vi "test tools list cache.vi"(8 "error in (no error)":errorcluster, 11 "server id":i32) -> (0 "error out":errorcluster, 3 "body":string)   [LabVIEW 2020, in "MCP Server tests.lvlib"]
doc: "Test 75: tools/list is answered from the cache and follows Add Tool.\n\nThe server builds the list of tools once and answers the following tools/list requests from Tool List Cache.vi (Cached Tool List.vi) until the tools of the server change.\n\n1. Two consecutive tools/list requests with the same id get exactly the same answer, with result.tools and without fake_tool_added_later.\n2. The second of the two, which is answered from the cache, takes less than 500 ms. The label of the assertion carries the measured time. Measured on LabVIEW 2026 with the 20 tools of this suite: 112 to 154 ms, most of it the HTTP round trip of two requests in a row.\n3. Add Tool.vi adds fake tool added later.vi to the running server; the next tools/list contains fake_tool_added_later, so the cache follows the tools.\n4. The tools/list after that gets the same answer again.\n\nThe added tool stays on the server of this test run; run this test after the tests that expect a fixed list of tools."
uses:
  MCP Server tests.lvlib
  de18a1eb-e5a6-43c2-9401-4d16a1e6fda1.vi
  a5e1876d-9ffb-455d-837e-6668acf3c3fd.vi
  <vilib>/JDP Science/JSONtext/Next JSON Value.vi
  <vilib>/JDP Science/JSONtext/String Subset.vi
  <vilib>/JDP Science/JSONtext/Parsing/Advance past next JSON Value (inlined COPY).vi
  <vilib>/JDP Science/JSONtext/Parsing/Advance past whitespace.vi
  <vilib>/JDP Science/JSONtext/Parsing/Advance past String.vi
  <vilib>/JDP Science/JSONtext/Parsing/Advance past Number.vi
  <vilib>/JDP Science/JSONtext/Parsing/Advance past Line Ending.vi
  <vilib>/JDP Science/JSONtext/Parsing/Parse Full Path or Item Name.vi
  <vilib>/JDP Science/JSONtext/Parsing/Advance past Array.vi
  <vilib>/JDP Science/JSONtext/Parsing/Advance past Object.vi
  <vilib>/JDP Science/JSONtext/support/Error Cluster From Code.vi
  <vilib>/JDP Science/JSONtext/Offset/Find Item Locations by Path.vi
  <vilib>/addons/_JKI Toolkits/Caraya/classes/Test/Test.lvclass
  <vilib>/JDP Science/JSONtext/JSONtext.lvlib
  <vilib>/addons/_JKI Toolkits/Caraya/classes/Assert/Assert.lvclass
  src/MCP Server/MCP Server.lvlib
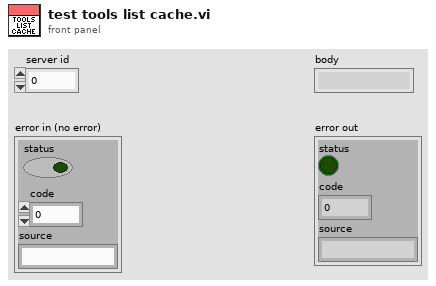
[diagram p1: front panel]
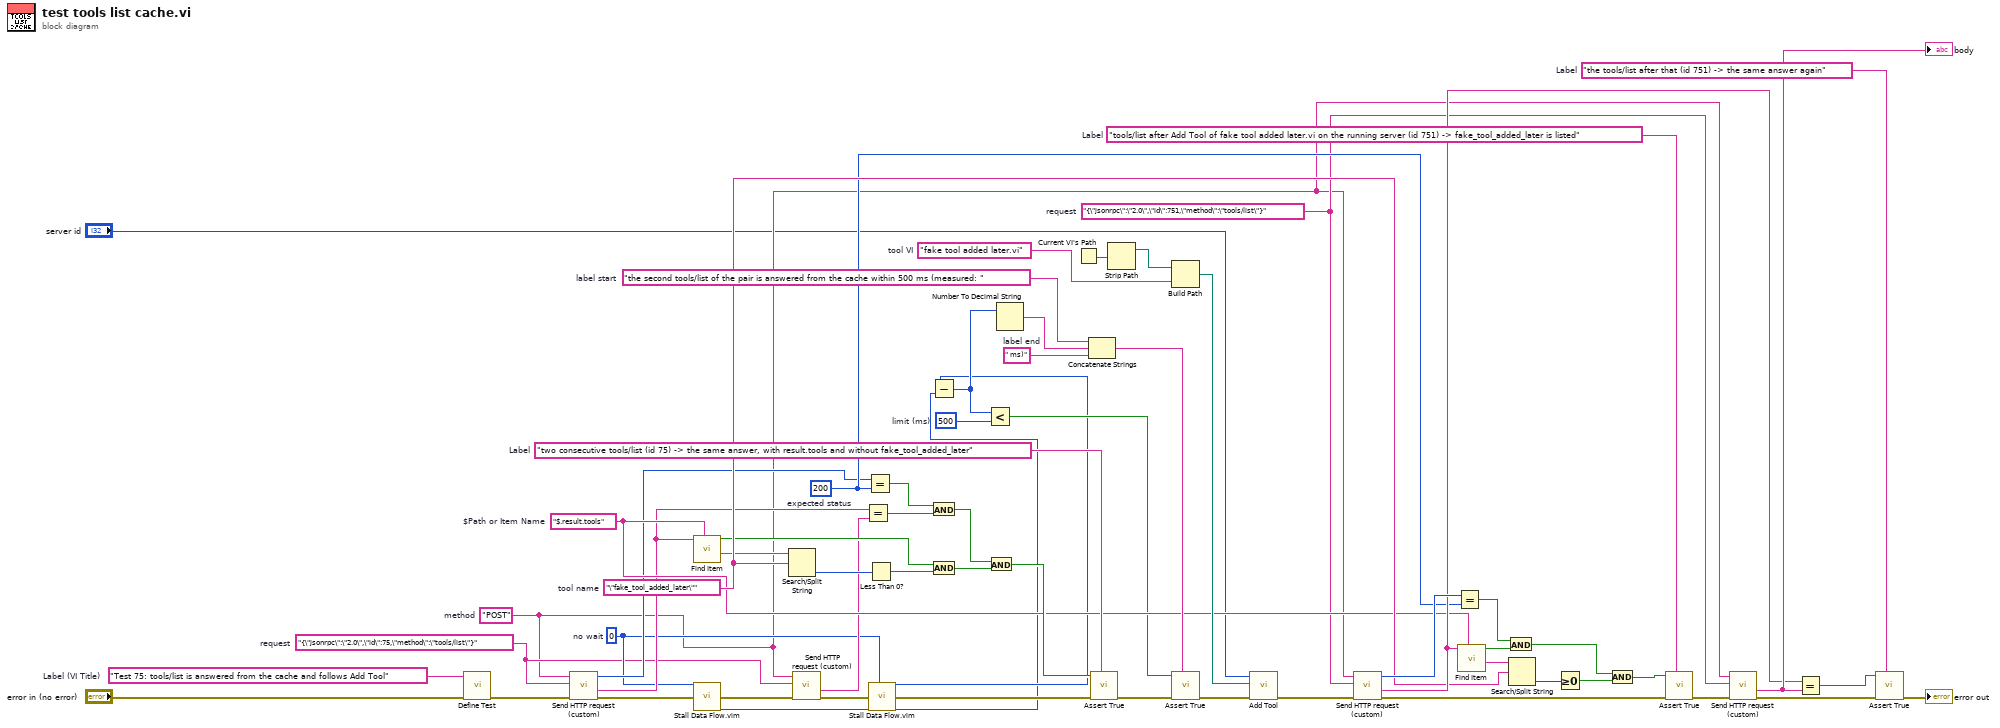
[diagram p0: block diagram]
diagram:
  w60 = "the tools/list after that (id 751) -> the same answer again"  # Label
  w55 = "tools/list after Add Tool of fake tool added later.vi on the running server (id 751) -> fake_tool_added_later is listed"  # Label
  w40 = "fake tool added later.vi"  # tool VI
  w37 = " ms)"  # label end
  w36 = "the second tools/list of the pair is answered from the cache within 500 ms (measured: "  # label start
  w33 = "two consecutive tools/list (id 75) -> the same answer, with result.tools and without fake_tool_added_later"  # Label
  w27 = "\"fake_tool_added_later\""  # tool name
  w24 = "$.result.tools"  # $Path or Item Name
  w21 = 200  # expected status
  w19 = u32 500  # limit (ms)
  w8 = 0  # no wait
  w7 = "{\"jsonrpc\":\"2.0\",\"id\":751,\"method\":\"tools/list\"}"  # request
  w6 = "{\"jsonrpc\":\"2.0\",\"id\":75,\"method\":\"tools/list\"}"  # request
  w5 = "POST"  # method
  w3 = "Test 75: tools/list is answered from the cache and follows Add Tool"  # Label (VI Title)
  n1 = call <vilib>:"Define Test.vi"("error in (no error)"="error in (no error)", "Label (VI Title)"=w3) -> ("error out"=w4:errorcluster)  [unwired: 8 in, 1 out]
  n2 = call "Send HTTP request (custom).vi"("error in (no error)"=w4, "request"=w6, "method"=w5) -> ("error out"=w9:errorcluster, "response"=w10:string, "status code"=w11:i32)  [unwired: 5 in, 1 out]
  n3 = call <vilib>:"Find Item.vi"("$Path or Item Name"=w24, "JSON"=w10) -> ("<JSON>"=w25:string, "Found"=w26:bool)  [unwired: 6 in, 2 out]
  n4 = call "Stall Data Flow.vim"("value in"=w9, "milliseconds to wait"=w8) -> ("millisecond timer value"=w12:u32, "value out"=w13:errorcluster)
  n5 = Search/Split String(string=w25, search string/char (-)=w27) -> (offset of match=w28:i32)  [unwired: 1 in, 2 out]
  n6 = call "Send HTTP request (custom).vi"("error in (no error)"=w13, "request"=w6, "method"=w5) -> ("error out"=w14:errorcluster, "response"=w15:string)  [unwired: 5 in, 2 out]
  n7 = Equal?(x=w10, y=w15) -> (x = y?=w23:bool)
  n8 = Equal?(x=w11, y=w21) -> (x = y?=w22:bool)
  n9 = Less Than 0?(x=w28) -> (x < 0?=w29:bool)
  n10 = call "Stall Data Flow.vim"("value in"=w14, "milliseconds to wait"=w8) -> ("millisecond timer value"=w16:u32, "value out"=w17:errorcluster)
  n11 = Subtract(x=w16, y=w12) -> (x-y=w18:u32)
  n12 = And(x=w22, y=w23) -> (x .and. y?=w30:bool)
  n13 = And(x=w26, y=w29) -> (x .and. y?=w31:bool)
  n14 = Less?(x=w18, y=w19) -> (x < y?=w20:bool)
  n15 = And(x=w30, y=w31) -> (x .and. y?=w32:bool)
  n16 = Number To Decimal String(number=w18) -> (decimal integer string=w35:string)  [unwired: 1 in]
  n17 = Current VI's Path() -> (path=w41:path)
  n18 = Concatenate Strings(w36, w35, w37) -> (w38:string)
  n19 = call <vilib>:"Assert True.vi"("Label"=w33, "error in (no error)"=w17, "True?"=w32) -> ("error out"=w34:errorcluster)  [unwired: 7 in, 1 out]
  n20 = Strip Path(path=w41) -> (stripped path=w42:path)  [unwired: 1 out]
  n21 = Build Path(base path=w42, name or relative path=w40) -> (appended path=w43:path)
  n22 = call <vilib>:"Assert True.vi"("Label"=w38, "error in (no error)"=w34, "True?"=w20) -> ("error out"=w39:errorcluster)  [unwired: 7 in, 1 out]
  n23 = call "Add Tool.vi"("error in (no error)"=w39, "vi path"=w43, "server id"="server id") -> ("error out"=w44:errorcluster)  [unwired: 7 in, 1 out]
  n24 = call "Send HTTP request (custom).vi"("error in (no error)"=w44, "request"=w7, "method"=w5) -> ("error out"=w45:errorcluster, "response"=w46:string, "status code"=w47:i32)  [unwired: 5 in, 1 out]
  n25 = Equal?(x=w47, y=w21) -> (x = y?=w48:bool)
  n26 = call <vilib>:"Find Item.vi"("$Path or Item Name"=w24, "JSON"=w46) -> ("<JSON>"=w49:string, "Found"=w50:bool)  [unwired: 6 in, 2 out]
  n27 = And(x=w48, y=w50) -> (x .and. y?=w53:bool)
  n28 = Search/Split String(string=w49, search string/char (-)=w27) -> (offset of match=w51:i32)  [unwired: 1 in, 2 out]
  n29 = Greater Or Equal To 0?(x=w51) -> (x >= 0?=w52:bool)
  n30 = And(x=w53, y=w52) -> (x .and. y?=w54:bool)
  n31 = call <vilib>:"Assert True.vi"("Label"=w55, "error in (no error)"=w45, "True?"=w54) -> ("error out"=w56:errorcluster)  [unwired: 7 in, 1 out]
  n32 = call "Send HTTP request (custom).vi"("error in (no error)"=w56, "request"=w7, "method"=w5) -> ("error out"=w57:errorcluster, "response"=w58:string)  [unwired: 5 in, 2 out]
  "body" <- w58
  n33 = Equal?(x=w46, y=w58) -> (x = y?=w59:bool)
  n34 = call <vilib>:"Assert True.vi"("Label"=w60, "error in (no error)"=w57, "True?"=w59) -> ("error out"=→"error out":errorcluster)  [unwired: 7 in, 1 out]
